vi "绘图-分段颜色-差分.vi"(7 "分段颜色":enum32{"蓝色", "红色"}(ring), 8 "基准索引":i32, 9 "光谱值":dbl[](array[numeric]), 11 "清空":bool) -> (3 "数组":dbl[][](array[numeric]))   [LabVIEW 2026, in "UI-无创.lvlib"]
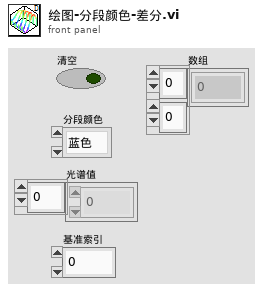
[diagram p1: front panel]
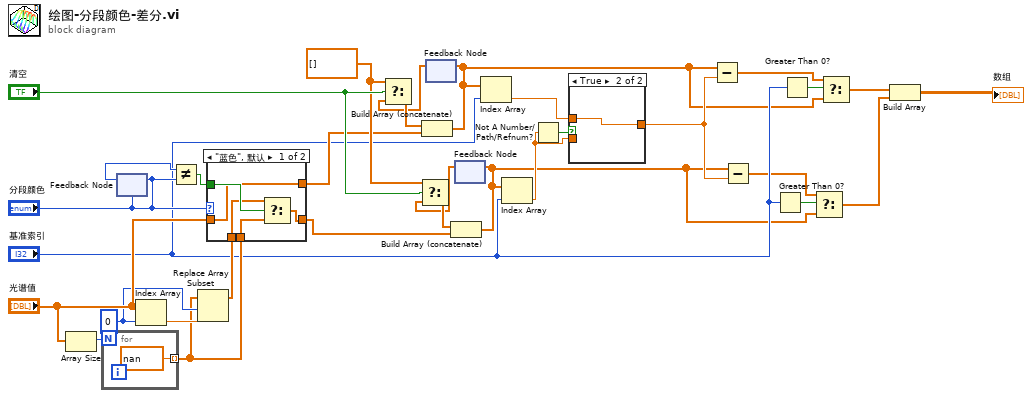
[diagram p0: block diagram]
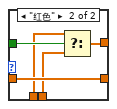
[diagram p2: hidden frame]
diagram:
  w12 = 0 ("索引")
  w21 = dbl[] []
  n1 = Array Size(array="光谱值") -> (size(s)=w15:i32)
  n2 = for {
    N: w15 -> [_]
    tunnel: [nan] -> w11 mode=indexing
  }
  n3 = feedback #1("分段颜色") -> (w20:enum32{"蓝色", "红色"})
  n4 = feedback-in #1("分段颜色") -> ()
  n5 = Index Array(array="光谱值", index=w12) -> (element=w13:dbl)
  n6 = Not Equal?(x=w20, y="分段颜色") -> (x != y?=w19:bool)
  n7 = Replace Array Subset(array=w11, new element=w13, index=w12) -> (w10:dbl[])
  n8 = case shown="\"蓝色\", 默认" "分段颜色" {
    tunnel: "光谱值" -> [w35 w41]
    tunnel: [w35 w40] -> w17
    tunnel: [w36 w41] -> w16
    tunnel: w19 -> [w37 w42]
    tunnel: w11 -> [w34 w39]
    tunnel: w10 -> [w33 w38]
    frame "蓝色", Default {
      n9 = Select(t=w33, s=w37, f=w34) -> (s? t:f=w36:dbl[])
    }
    frame "红色" {
      n10 = Select(t=w38, s=w42, f=w39) -> (s? t:f=w40:dbl[])
    }
  }
  n11 = feedback #2() -> (w22:dbl[])  [unwired: 1 in]
  n12 = Select(t=w21, s="清空", f=w22) -> (s? t:f=w23:dbl[])
  n13 = Build Array (concatenate)(w23, w17) -> (w5:dbl[])
  n14 = feedback-in #2(w5) -> ()
  n15 = feedback #3() -> (w24:dbl[])  [unwired: 1 in]
  n16 = Select(t=w21, s="清空", f=w24) -> (s? t:f=w25:dbl[])
  n17 = Build Array (concatenate)(w25, w16) -> (w2:dbl[])
  n18 = feedback-in #3(w2) -> ()
  n19 = Index Array(array=w5, index="基准索引") -> (element=w29:dbl)
  n20 = Index Array(array=w2, index="基准索引") -> (element=w30:dbl)
  n21 = Not A Number/Path/Refnum?(number/path/refnum=w30) -> (NaN/Path/Refnum?=w28:bool)
  n22 = case shown="True" w28 {
    tunnel: w29 -> [_ w44]
    tunnel: w30 -> [w43 _]
    tunnel: [w43 w44] -> w31
    frame False {
    }
    frame True {
    }
  }
  n23 = Subtract(x=w5, y=w31) -> (x-y=w6:dbl[])
  n24 = Subtract(x=w2, y=w31) -> (x-y=w3:dbl[])
  n25 = Greater Than 0?(x="基准索引") -> (x > 0?=w9:bool)
  n26 = Greater Than 0?(x="基准索引") -> (x > 0?=w8:bool)
  n27 = Select(t=w3, s=w9, f=w2) -> (s? t:f=w1:dbl[])
  n28 = Select(t=w6, s=w8, f=w5) -> (s? t:f=w4:dbl[])
  n29 = Build Array(w4, w1) -> (→"数组":dbl[][])
